vi "Multicast Endpoint.vi"(8 "error in (no error)":errorcluster, 11 "Group in":refnum<class "Group Config.lvclass">) -> (0 "error out":errorcluster, 2 "Multicast Endpoint":T1, 3 "Group out":refnum<class "Group Config.lvclass">)   [LabVIEW 2020, in "VolatusConfig.lvlib" / "Group Config.lvclass"]
uses:
  Group Config.lvclass
  C:/dev/lv20CE/relink/lv-volatus/VolatusConfig/VolatusConfigElement/VolatusConfigElement.lvclass
  lv-vecto/VectoConfig/Endpoint.ctl
  VolatusConfigElement/VolatusConfigElement.lvclass/VolatusConfigElement.ctl
  Group Config.lvclass/Group Config.ctl
  lv-cdm/CDM-Config/Config Element/Config Element.lvclass
  VolatusConfigElement/VolatusConfigElement.lvclass
  lv-vecto/VectoConfig/VectoConfig.lvlib
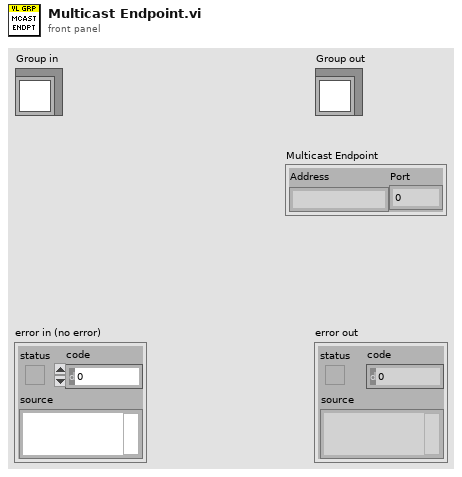
[diagram p1: front panel]
types:
  T1 = typedef "VectoConfig.lvlib/Endpoint.ctl" = cluster{"Address":string, "Port":u16}
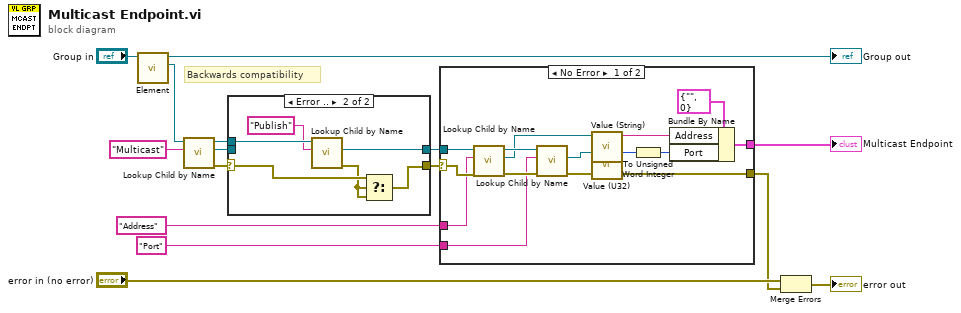
[diagram p0: block diagram]
diagram:
  # "Backwards compatibility"
  n1 = call "Element.vi"("VolatusConfigElement in"="Group in") -> ("Element"=w6:refnum<class "Config Element.lvclass">, "VolatusConfigElement out"=→"Group out":refnum<class "Group Config.lvclass">)  [unwired: 9 in]
  n2 = call "Lookup Child by Name.vi"("Name"="Multicast", "Config Element in"=w6) -> ("error out"=w5:errorcluster, "Child"=w3:refnum<class "Config Element.lvclass">, "Config Element out"=w4:refnum<class "Config Element.lvclass">)  [unwired: 6 in, 1 out]
  n3 = case shown="Error .." w5 {
    selector: w5 -> [w16 w20]
    tunnel: w4 -> [_ w23]
    tunnel: w3 -> [w17 _]
    tunnel: [w17 w22] -> w2
    tunnel: [w16 w18] -> w1
    frame No Error {
    }
    frame Error {
      n4 = call "Lookup Child by Name.vi"("Name"="Publish", "Config Element in"=w23) -> ("error out"=w19:errorcluster, "Child"=w22:refnum<class "Config Element.lvclass">)  [unwired: 6 in, 2 out]
      n5 = Select(t=w20, s=w19, f=w19) -> (s? t:f=w18:errorcluster)
    }
  }
  n6 = case shown="No Error" w1 {
    selector: w1 -> [w35 _]
    tunnel: w2 -> [w36 _]
    tunnel: "Address" ("Name") -> [w34 _]
    tunnel: "Port" ("Name") -> [w32 _]
    tunnel: [w25 _] -> w9
    tunnel: [w24 _] -> w8
    frame No Error {
      n7 = call "Lookup Child by Name.vi"("error in (no error)"=w35, "Name"=w34, "Config Element in"=w36) -> ("error out"=w37:errorcluster, "Child"=w26:refnum<class "Config Element.lvclass">, "Config Element out"=w33:refnum<class "Config Element.lvclass">)  [unwired: 5 in, 1 out]
      n8 = call "Lookup Child by Name.vi"("error in (no error)"=w37, "Name"=w32, "Config Element in"=w33) -> ("error out"=w25:errorcluster, "Child"=w30:refnum<class "Config Element.lvclass">)  [unwired: 5 in, 2 out]
      n9 = call "Value (String).vi"("Config Element in"=w26) -> ("String Value"=w27:string)  [unwired: 9 in, 1 out]
      n10 = call "Value (U32).vi"("Config Element in"=w30) -> ("U32 Value"=w29:u32)  [unwired: 9 in, 1 out]
      n11 = To Unsigned Word Integer(number=w29) -> (unsigned 16bit integer=w28:u16)
      n12 = Bundle By Name(cluster=T1 {"Address"="", "Port"=0} ("Endpoint"), "Address"=w27, "Port"=w28) -> (w24:T1)
    }
    frame Error {
      # "Doesn't have publish config which is fine, it just won't be published."
    }
  }
  "Multicast Endpoint" <- w8
  n13 = Merge Errors("error in (no error)", w9) -> (→"error out":errorcluster)
